vi "_LatchTest.vi"(0 "VI Reference In":refnum<vi>, 5 "Subpanel Details":string, 11 "error in":errorcluster) -> (4 "VI Reference Out":refnum<vi>, 15 "error out":errorcluster)   [LabVIEW 2016, in "SubpanelTests.lvlib"]
doc: "Boolean Latch Test"
uses:
  SubpanelTests.lvlib
  APIs/Stimulus/ControlValue/ValueSignalLatchBooleanString.vi
  APIs/Assert/AssertControlValue/Equal.vi
  <vilib>/addons/_JKI Toolkits/Caraya/classes/Test/Test.lvclass
  Drona.lvlib
  APIs/Assert/AssertControlValue/AssertControlValue.lvlib
  APIs/Stimulus/ControlValue/ControlValue.lvlib
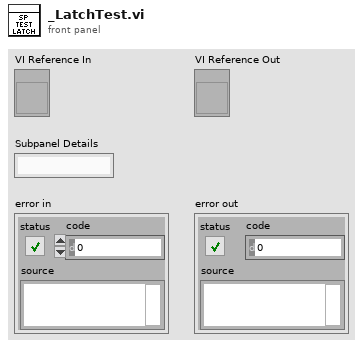
[diagram p1: front panel]
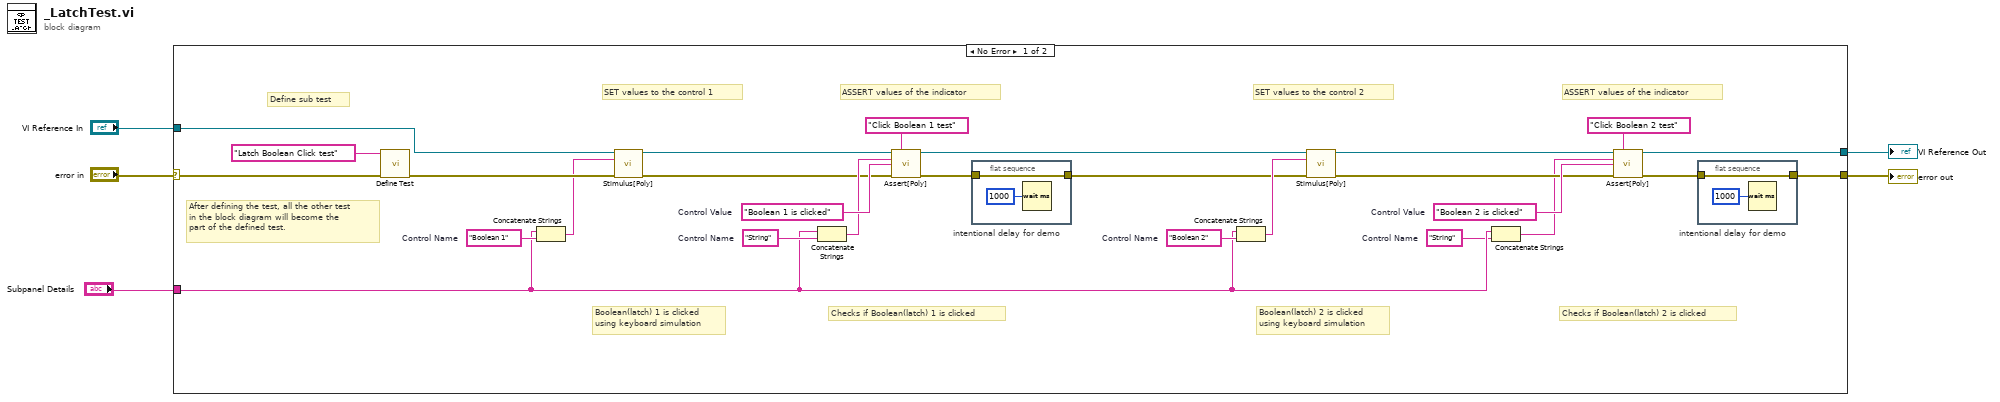
[diagram p0: block diagram]
diagram:
  n1 = case shown="No Error" "error in" {
    selector: "error in" -> [w20 w37]
    tunnel: "VI Reference In" -> [w22 w38]
    tunnel: [w21 w38] -> w4
    tunnel: "Subpanel Details" -> [w13 _]
    tunnel: [w6 w37] -> w1
    frame No Error {
      w12 = "String"  # Control Name
      w27 = "Boolean 2 is clicked"  # Control Value
      w15 = "Boolean 2"  # Control Name
      w17 = "String"  # Control Name
      w30 = "Boolean 1 is clicked"  # Control Value
      w19 = "Boolean 1"  # Control Name
      # "Checks if Boolean(latch) 2 is clicked"
      # "ASSERT values of the indicator"
      # "Boolean(latch) 2 is clicked\nusing keyboard simulation"
      # "SET values to the control 2"
      # "Checks if Boolean(latch) 1 is clicked"
      # "ASSERT values of the indicator"
      # "Boolean(latch) 1 is clicked\nusing keyboard simulation"
      # "SET values to the control 1"
      # "After defining the test, all the other test\nin the block diagram will become the \npart of the defined test."
      # "Define sub test"
      n2 = call <vilib>:"Define Test.vi"("error in (no error)"=w20, "Label (VI Title)"="Latch Boolean Click test") -> ("error out"=w23:errorcluster)  [unwired: 8 in, 1 out]
      n3 = Concatenate Strings(w13, w19) -> (w18:string)
      n4 = call-poly "Stimulus[Poly].vi"("VI Reference In"=w22, "Control Path"=w18, "error in"=w23) -> ("VI Reference Out"=w31:refnum<vi>, "error out"=w10:errorcluster)  [unwired: 11 in]
      n5 = Concatenate Strings(w13, w17) -> (w16:string)
      n6 = call-poly "Assert[Poly].vi"("VI Reference In"=w31, "Test Label"="Click Boolean 1 test" ("Label (VI Title)"), "Control Path"=w16, "Control Value"=w30, "Error In"=w10) -> ("VI Reference Out"=w26:refnum<vi>, "Error Out"=w9:errorcluster)  [unwired: 8 in, 1 out]
      n7 = flat-sequence "intentional delay for demo" {
        tunnel: w9 -> [w35]
        tunnel: [w35] -> w8
        frame #0 {
          n8 = Wait (ms)(milliseconds to wait=u32 1000) -> ()  [unwired: 1 out]
        }
      }
      n9 = Concatenate Strings(w13, w15) -> (w14:string)
      n10 = call-poly "Stimulus[Poly].vi"("VI Reference In"=w26, "Control Path"=w14, "error in"=w8) -> ("VI Reference Out"=w24:refnum<vi>, "error out"=w25:errorcluster)  [unwired: 11 in]
      n11 = Concatenate Strings(w13, w12) -> (w11:string)
      n12 = call-poly "Assert[Poly].vi"("VI Reference In"=w24, "Test Label"="Click Boolean 2 test" ("Label (VI Title)"), "Control Path"=w11, "Control Value"=w27, "Error In"=w25) -> ("VI Reference Out"=w21:refnum<vi>, "Error Out"=w7:errorcluster)  [unwired: 8 in, 1 out]
      n13 = flat-sequence "intentional delay for demo" {
        tunnel: w7 -> [w33]
        tunnel: [w33] -> w6
        frame #0 {
          n14 = Wait (ms)(milliseconds to wait=u32 1000) -> ()  [unwired: 1 out]
        }
      }
    }
    frame Error {
    }
  }
  "error out" <- w1
  "VI Reference Out" <- w4
